vi "Room_Change.vi"(0 "State":T1={"Tick"=0, "Phase"=0, "PhaseTicks"=0, "Level"=1, "Room"=0, "X10"=0, "Y10"=0, "VY10"=0, "Mode"=0, "Facing"=0, "Run"=0, "Vert"=0, "StandY"=0, "EntryX10"=0, "EntryY10"=0, "EntryMode"=0, "Lives"=4, "Score"=0, "NextLife"=10000, "KeyR"=0, "KeyB"=0, "KeyY"=0, "Torch"=FALSE, "FloorPhase"=0, "Dead"=FALSE, "LevelStart"=FALSE, "Quit"=FALSE, "Sound"=0, "Seed"=12345, "DemoStep"=0, "Tiles"=[], "World"=[], "Enemies"=[], "Highscores"=[], "Name"=[0, 0, 0], "Cursor"=0}, 11 "error in":errorcluster) -> (4 "State out":T1={"Tick"=0, "Phase"=0, "PhaseTicks"=0, "Level"=1, "Room"=0, "X10"=0, "Y10"=0, "VY10"=0, "Mode"=0, "Facing"=0, "Run"=0, "Vert"=0, "StandY"=0, "EntryX10"=0, "EntryY10"=0, "EntryMode"=0, "Lives"=4, "Score"=0, "NextLife"=10000, "KeyR"=0, "KeyB"=0, "KeyY"=0, "Torch"=FALSE, "FloorPhase"=0, "Dead"=FALSE, "LevelStart"=FALSE, "Quit"=FALSE, "Sound"=0, "Seed"=12345, "DemoStep"=0, "Tiles"=[], "World"=[], "Enemies"=[], "Highscores"=[], "Name"=[0, 0, 0], "Cursor"=0}, 6 "Changed":bool, 15 "error out":errorcluster)   [LabVIEW 2020, in "GH_Engine.lvlib"]
doc: "Changes the room when the middle of Claude leaves the playfield: left/right to the neighbour in the same depth, up/down to the room above/below. The tiles of the old room (gold taken, doors opened) are stored in World, the new room comes from World, its enemies start again (Enemies_Init). The position moves by one room size, the fall height carries over, the arrival is the new restart point. Without a room above, Claude cannot leave the top of the playfield."
uses:
  GH_Engine.lvlib
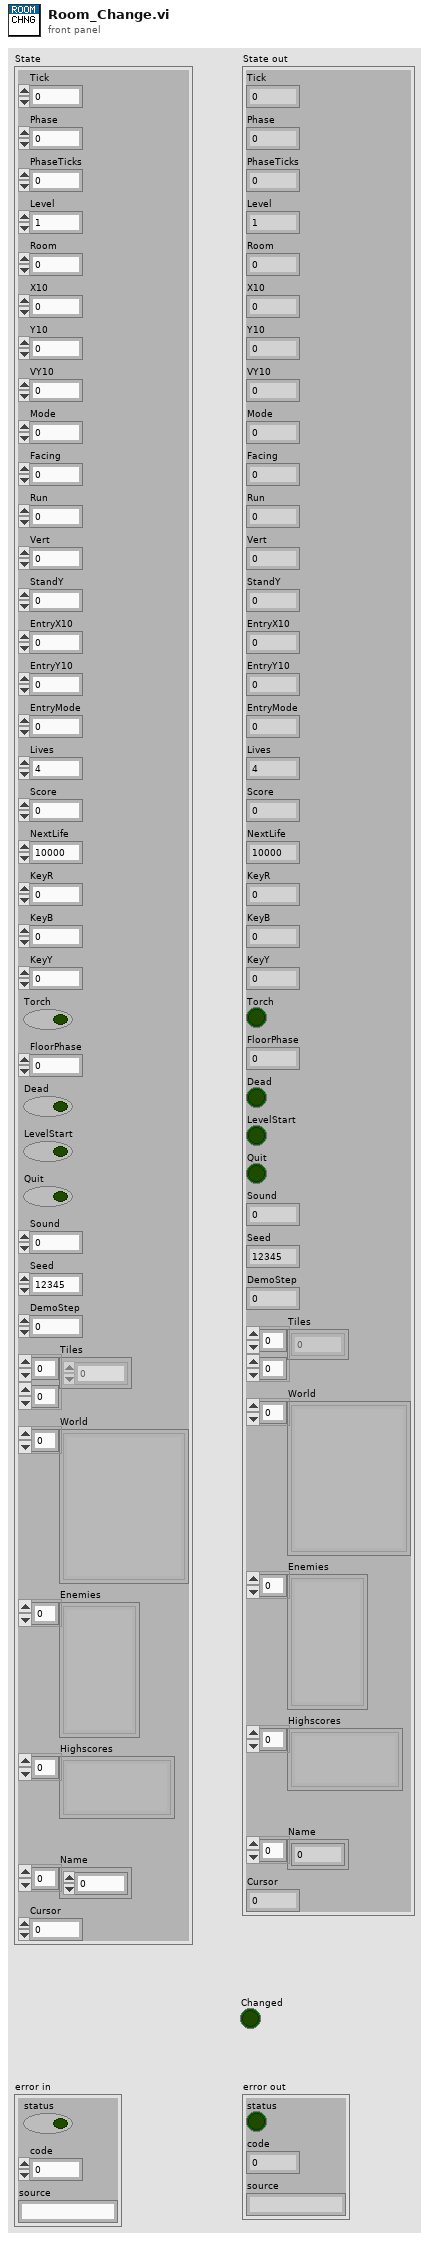
[diagram p1: front panel]
types:
  T1 = cluster{"Tick":u32, "Phase":i32, "PhaseTicks":i32, "Level":i32, "Room":i32, "X10":i32, "Y10":i32, "VY10":i32, "Mode":i32, "Facing":i32, "Run":i32, "Vert":i32, "StandY":i32, "EntryX10":i32, "EntryY10":i32, "EntryMode":i32, "Lives":i32, "Score":i32, "NextLife":i32, "KeyR":i32, "KeyB":i32, "KeyY":i32, "Torch":bool, "FloorPhase":i32, "Dead":bool, "LevelStart":bool, "Quit":bool, "Sound":i32, "Seed":u32, "DemoStep":i32, "Tiles":u8[][], "World":cluster{"ID":string, "Depth":i32, "Column":i32, "Tiles":u8[][]}[], "Enemies":cluster{"Kind":i32, "X10":i32, "Y10":i32, "Dir":i32, "Mode":i32}[], "Highscores":cluster{"Score":i32, "Name":string}[], "Name":i32[], "Cursor":i32}
  T2 = cluster{"ID":string, "Depth":i32, "Column":i32, "Tiles":u8[][]}[]
  T3 = cluster{"ID":string, "Depth":i32, "Column":i32, "Tiles":u8[][]}
  T4 = cluster{"Kind":i32, "X10":i32, "Y10":i32, "Dir":i32, "Mode":i32}[]
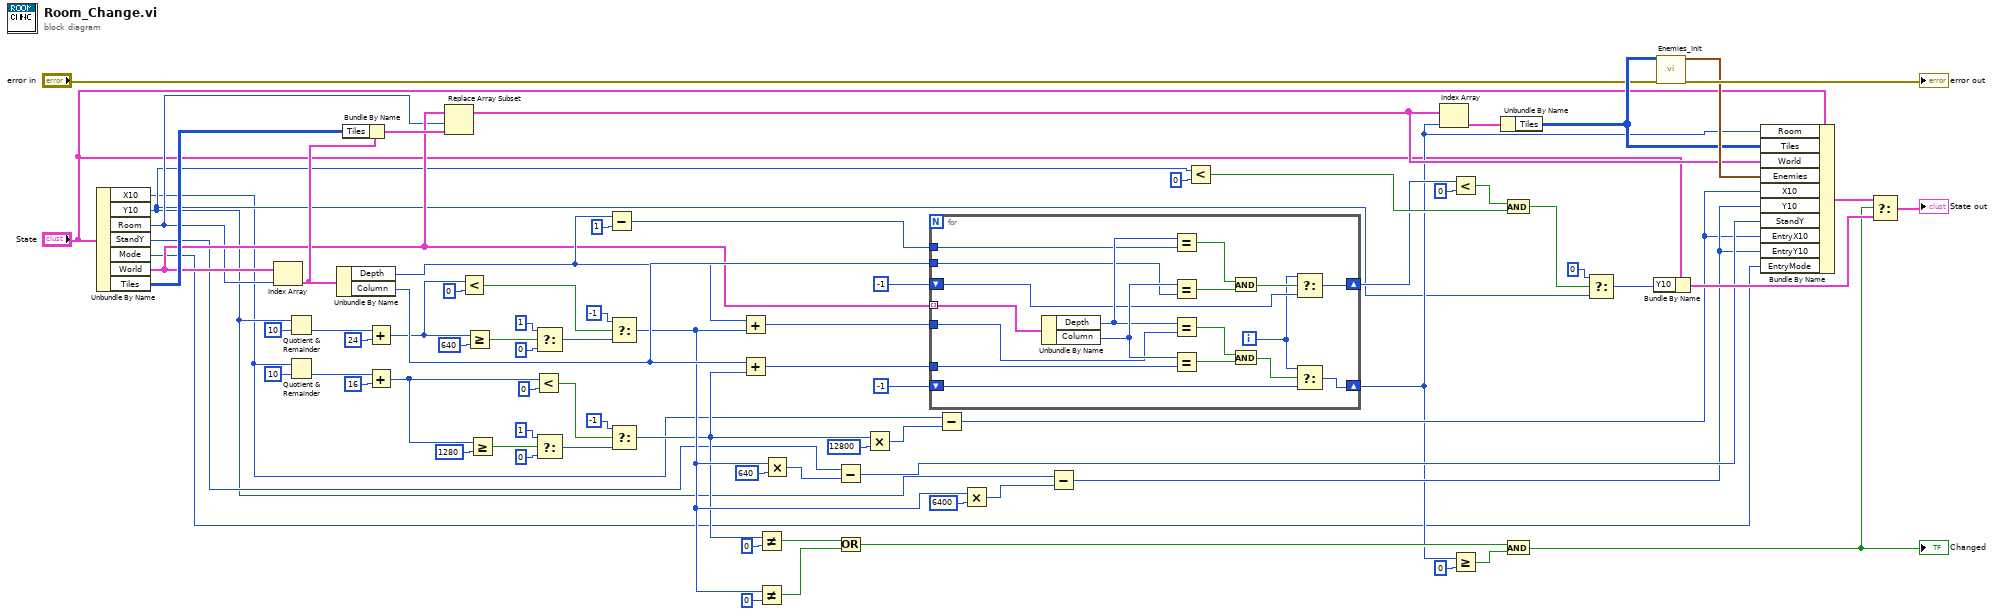
[diagram p0: block diagram]
diagram:
  n1 = Unbundle By Name("State") -> ("X10"=w3:i32, "Y10"=w4:i32, "Room"=w5:i32, "StandY"=w6:i32, "Mode"=w7:i32, "World"=w8:T2, "Tiles"=w9:u8[][])
  n2 = Index Array(array=w8, index=w5) -> (element=w36:T3)
  n3 = Quotient & Remainder(x=w4, y=10) -> (floor(x/y)=w15:i32)  [unwired: 1 out]
  n4 = Quotient & Remainder(x=w3, y=10) -> (floor(x/y)=w11:i32)  [unwired: 1 out]
  n5 = Unbundle By Name(w36) -> ("Depth"=w37:i32, "Column"=w38:i32)
  n6 = Bundle By Name(cluster=w36, "Tiles"=w9) -> (w55:T3)
  n7 = Add(x=w15, y=24) -> (x+y=w17:i32)
  n8 = Add(x=w11, y=16) -> (x+y=w13:i32)
  n9 = Replace Array Subset(array=w8, new element=w55, index=w5) -> (w56:T2)
  n10 = Less?(x=w17, y=0) -> (x < y?=w28:bool)
  n11 = Greater Or Equal?(x=w17, y=640) -> (x >= y?=w31:bool)
  n12 = Greater Or Equal?(x=w13, y=1280) -> (x >= y?=w22:bool)
  n13 = Less?(x=w13, y=0) -> (x < y?=w19:bool)
  n14 = Select(t=1, s=w31, f=0) -> (s? t:f=w34:i32)
  n15 = Select(t=1, s=w22, f=0) -> (s? t:f=w25:i32)
  n16 = Subtract(x=w37, y=1) -> (x-y=w42:i32)
  n17 = Select(t=-1, s=w28, f=w34) -> (s? t:f=w35:i32)
  n18 = Select(t=-1, s=w19, f=w25) -> (s? t:f=w26:i32)
  n19 = Add(x=w37, y=w35) -> (x+y=w39:i32)
  n20 = Add(x=w38, y=w26) -> (x+y=w40:i32)
  n21 = Not Equal?(x=w26, y=0) -> (x != y?=w48:bool)
  n22 = Not Equal?(x=w35, y=0) -> (x != y?=w50:bool)
  n23 = Multiply(x=w35, y=640) -> (x*y=w68:i32)
  n24 = Subtract(x=w6, y=w68) -> (x-y=w69:i32)
  n25 = Or(x=w48, y=w50) -> (x .or. y?=w51:bool)
  n26 = Multiply(x=w26, y=12800) -> (x*y=w62:i32)
  n27 = for {
    shift-right: [w87] -> w45
    shift-left: -1 -> [w86]
    shift-right: [w89] -> w46
    shift-left: -1 -> [w88]
    tunnel: w8 -> [w81] mode=indexing
    tunnel: w38 -> [w85]
    tunnel: w42 -> [w84]
    tunnel: w39 -> [w82]
    tunnel: w40 -> [w83]
    i -> [w80]
    n28 = Unbundle By Name(w81) -> ("Depth"=w90:i32, "Column"=w91:i32)
    n29 = Equal?(x=w90, y=w84) -> (x = y?=w95:bool)
    n30 = Equal?(x=w91, y=w85) -> (x = y?=w96:bool)
    n31 = Equal?(x=w90, y=w82) -> (x = y?=w92:bool)
    n32 = Equal?(x=w91, y=w83) -> (x = y?=w93:bool)
    n33 = And(x=w95, y=w96) -> (x .and. y?=w97:bool)
    n34 = And(x=w92, y=w93) -> (x .and. y?=w94:bool)
    n35 = Select(t=w80, s=w97, f=w88) -> (s? t:f=w89:i32)
    n36 = Select(t=w80, s=w94, f=w86) -> (s? t:f=w87:i32)
  }
  n37 = Subtract(x=w3, y=w62) -> (x-y=w63:i32)
  n38 = Multiply(x=w35, y=6400) -> (x*y=w65:i32)
  n39 = Subtract(x=w4, y=w65) -> (x-y=w66:i32)
  n40 = Less?(x=w4, y=0) -> (x < y?=w74:bool)
  n41 = Index Array(array=w56, index=w45) -> (element=w57:T3)
  n42 = Less?(x=w46, y=0) -> (x < y?=w72:bool)
  n43 = Greater Or Equal?(x=w45, y=0) -> (x >= y?=w53:bool)
  n44 = Unbundle By Name(w57) -> ("Tiles"=w58:u8[][])
  n45 = And(x=w72, y=w74) -> (x .and. y?=w75:bool)
  n46 = And(x=w51, y=w53) -> (x .and. y?=w54:bool)
  "Changed" <- w54
  n47 = Select(t=0, s=w75, f=w4) -> (s? t:f=w77:i32)
  n48 = Bundle By Name(cluster="State", "Y10"=w77) -> (w78:T1)
  n49 = call "Enemies_Init.vi"("Tiles"=w58, "error in"="error in") -> ("Enemies"=w59:T4, "error out"=→"error out":errorcluster)  [unwired: 12 in]
  n50 = Bundle By Name(cluster="State", "Room"=w45, "Tiles"=w58, "World"=w56, "Enemies"=w59, "X10"=w63, "Y10"=w66, "StandY"=w69, "EntryX10"=w63, "EntryY10"=w66, "EntryMode"=w7) -> (w70:T1)
  n51 = Select(t=w70, s=w54, f=w78) -> (s? t:f=→"State out":T1)
